vi "VI_LV5_plasticnakutija.vi"() -> ()   [LabVIEW 2013]
panel:
  out "Izmjerena vrijednost":dynamicdata(graph)
  out "Nelinearizirana vrijednost":dbl
  in  "Pocet 4":bool
  in  "Zavrsit 4":bool
  in  "Broj uzoraka po semplu":dbl
  in  "Frekvencija":dbl
  out "Generisani signal":dynamicdata(graph)
  out "Prikuplljeni podaci":dynamicdata(graph)
  out "Linearizirana vrijednost":dbl
  # "Napon"
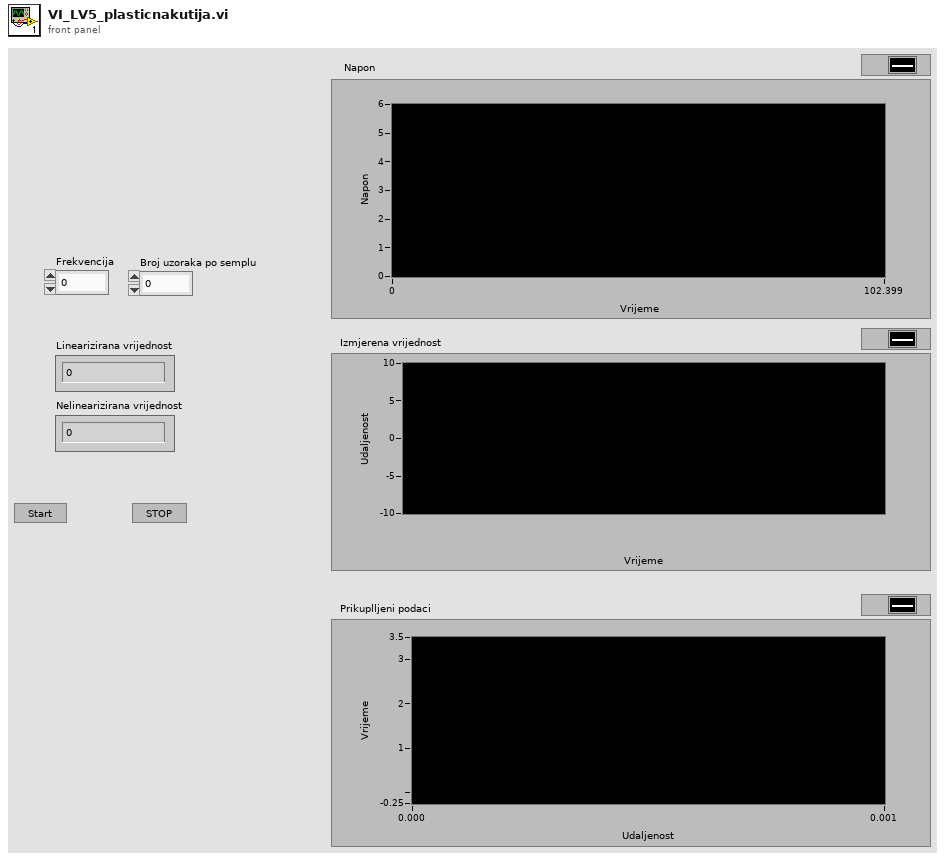
[diagram p1: front panel]
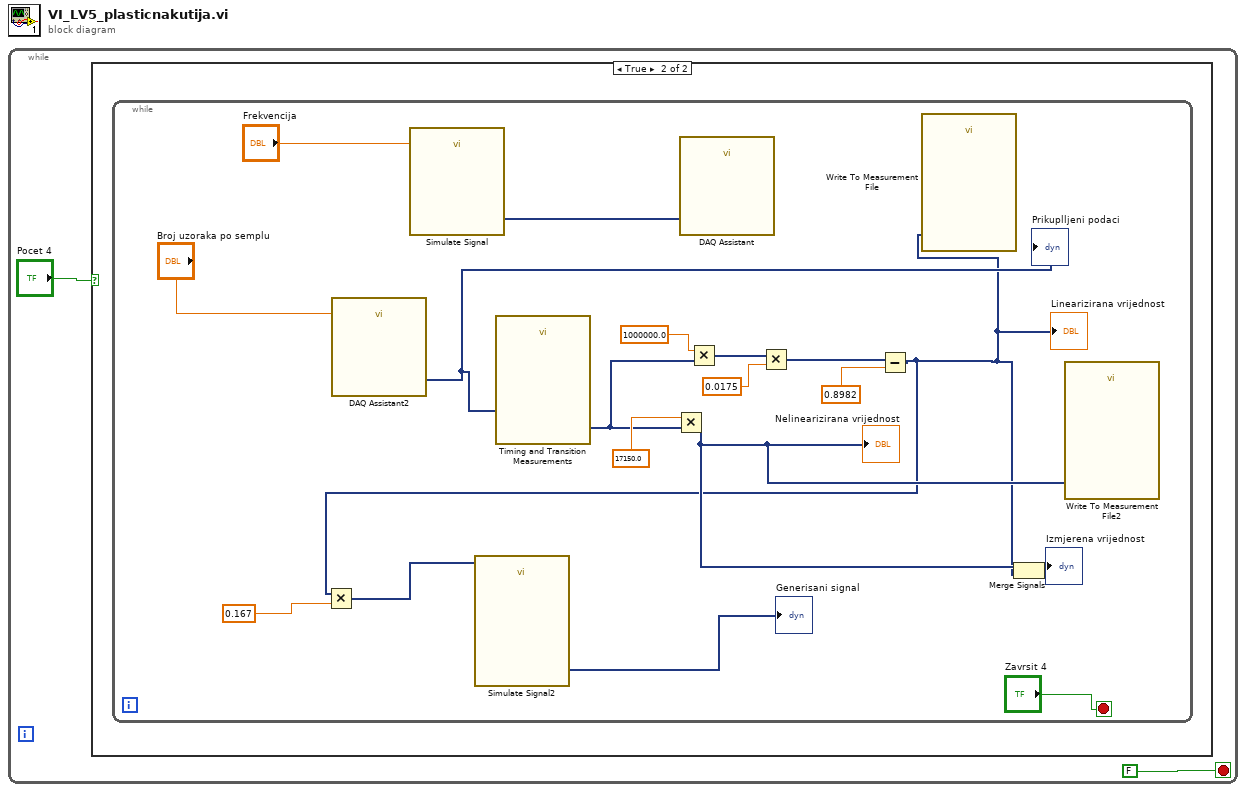
[diagram p0: block diagram]
diagram:
  n1 = while {
    stop <- FALSE stop-if-true
    n2 = case shown="True" "Pocet 4" {
      frame False {
      }
      frame True {
        n3 = while {
          stop <- "Zavrsit 4" stop-if-true
          n4 = call "DAQ Assistant2"("number of samples"="Broj uzoraka po semplu") -> ("data"=w19:dynamicdata)  [unwired: 16 in, 2 out]
          "Prikuplljeni podaci" <- w19
          n5 = call "Simulate Signal"("Frequency"="Frekvencija") -> ("Square"=w20:dynamicdata)  [unwired: 13 in, 1 out]
          n6 = call "Timing and Transition Measurements"("Signals"=w19) -> ("Duration"=w8:dynamicdata)  [unwired: 9 in, 1 out]
          n7 = Multiply(x=17150.0, y=w8) -> (x*y=w10:dynamicdata)
          "Nelinearizirana vrijednost" <- w10
          n8 = call "DAQ Assistant"("data"=w20) -> ()  [unwired: 16 in, 3 out]
          n9 = Multiply(x=1000000.0, y=w8) -> (x*y=w6:dynamicdata)
          n10 = Multiply(x=w6, y=0.0175 ("x")) -> (x*y=w4:dynamicdata)
          n11 = Subtract(x=w4, y=0.8982 ("x")) -> (x-y=w3:dynamicdata)
          "Linearizirana vrijednost" <- w3
          n12 = Multiply(x=w3, y=0.167 ("x")) -> (x*y=w17:dynamicdata)
          n13 = call "Simulate Signal2"("Offset"=w17) -> ("DC"=→"Generisani signal":dynamicdata)  [unwired: 13 in, 1 out]
          n14 = call "Write To Measurement File"("Signals"=w3) -> ()  [unwired: 16 in, 3 out]
          n15 = Merge Signals(w10, w3) -> (→"Izmjerena vrijednost":dynamicdata)
          n16 = call "Write To Measurement File2"("Signals"=w10) -> ()  [unwired: 16 in, 3 out]
        }
      }
    }
  }
